vi "Add ECAT Slave from Config.vi"(8 "error in (no error)":errorcluster, 10 "Section Ptr":T4 format="%.0x", 11 "Slave":T1) -> (0 "error out":errorcluster)   [LabVIEW 2020, in "SEECD System Explorer.lvlib"]
uses:
  SEECD System Explorer.lvlib
  <vilib>/NI VeriStand/Custom Device API/Custom Device Item Ref.ctl
  Type Defs/Host - Slave.ctl
  Type Defs/Host - Module.ctl
  Type Defs/IOV Container Contents.ctl
  Includes/Modules.lvlibp/RSI Module/Slot Settings.ctl
  Includes/Modules.lvlibp/RSI Module/Module Models.ctl
  Shared/Globals/Scan Engine GUIDs.vi
  Shared/Globals/String Constants.vi
  Shared/Globals/Property Strings.vi
  Includes/Modules.lvlibp/RSI Module/Class Property Strings.vi
  Includes/Modules.lvlibp/RSI Module/RSI Module.lvclass
  Includes/Modules.lvlibp/RemIO Module/RemIO Module.lvclass
  Shared/SEECD Shared.lvlib
  <vilib>/NI VeriStand/Custom Device API/Custom Device API.lvlib
  Includes/Modules.lvlibp
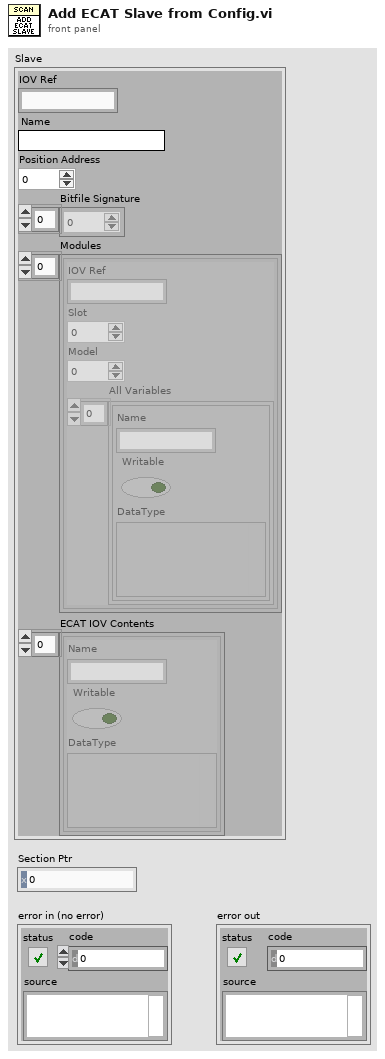
[diagram p1: front panel]
types:
  T1 = typedef "SEECD System Explorer.lvlib/Host - Slave.ctl" = cluster{"IOV Ref":string, "Name":string, "Position Address":u16, "Bitfile Signature":u8[], "Modules":T2[], "ECAT IOV Contents":T3[]}
  T2 = typedef "SEECD System Explorer.lvlib/Host - Module.ctl" = cluster{"IOV Ref":string, "Slot":u32, "Model":u32, "All Variables":T3[]}
  T3 = typedef "SEECD System Explorer.lvlib/IOV Container Contents.ctl" = cluster{"Name":string, "Writable":bool, "DataType":variant}
  T4 = typedef "Custom Device API.lvlib/Custom Device Item Ref.ctl" = u64
  T5 = typedef "Modules.lvlibp/RSI Module.lvclass/Slot Settings.ctl" = cluster{"Slot":u32, "EtherCAT?":bool}
  T6 = typedef "Modules.lvlibp/RSI Module.lvclass/Module Models.ctl" = enum16{"Empty", "NI 9201", "NI 9203", "NI 9205", "NI 9206", "NI 9207", "NI 9208", "NI 9209", "NI 9210", "NI 9211", "NI 9212", "NI 9213", "NI 9214", "NI 9215", "NI 9216", "NI 9217", "NI 9219", "NI 9220", "NI 9221", "NI 9222", "NI 9223", "NI 9224", "NI 9225", "NI 9226", "NI 9227", "NI 9228", "NI 9229", "NI 9233", "NI 9234", "NI 9235", "NI 9236", "NI 9237", "NI 9239", "NI 9242", "NI 9244", "NI 9253", "NI 9263", "NI 9264", "NI 9265", "NI 9266", "NI 9269", "NI 9344", "NI 9350", "NI 9375", "NI 9401", "NI 9402", "NI 9403", "NI 9411", "NI 9421", "NI 9422", "NI 9423", "NI 9425", "NI 9426", "NI 9435", "NI 9436", "NI 9437", "NI 9472", "NI 9474", "NI 9475", "NI 9476", "NI 9477", "NI 9478", "NI 9481", "NI 9482", "NI 9485"}
  T7 = typedef "Modules.lvlibp/Custom Device API.lvlib/Custom Device Item Ref.ctl" = u64
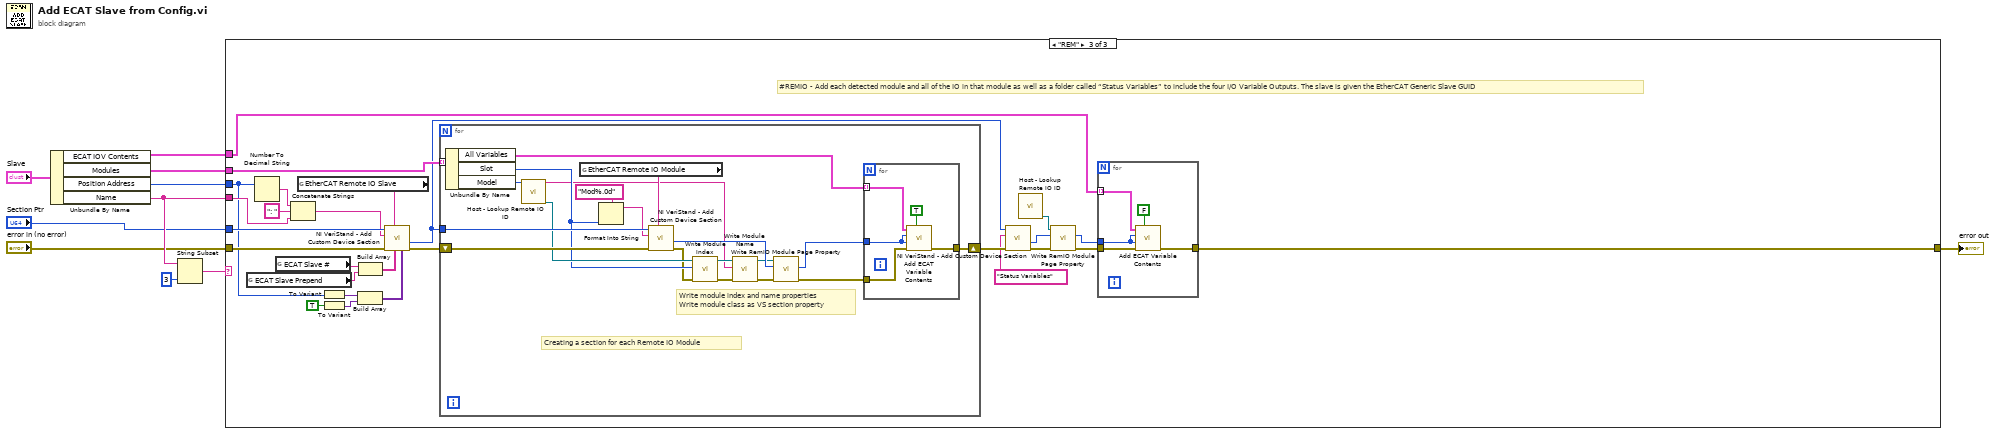
[diagram p0: block diagram]
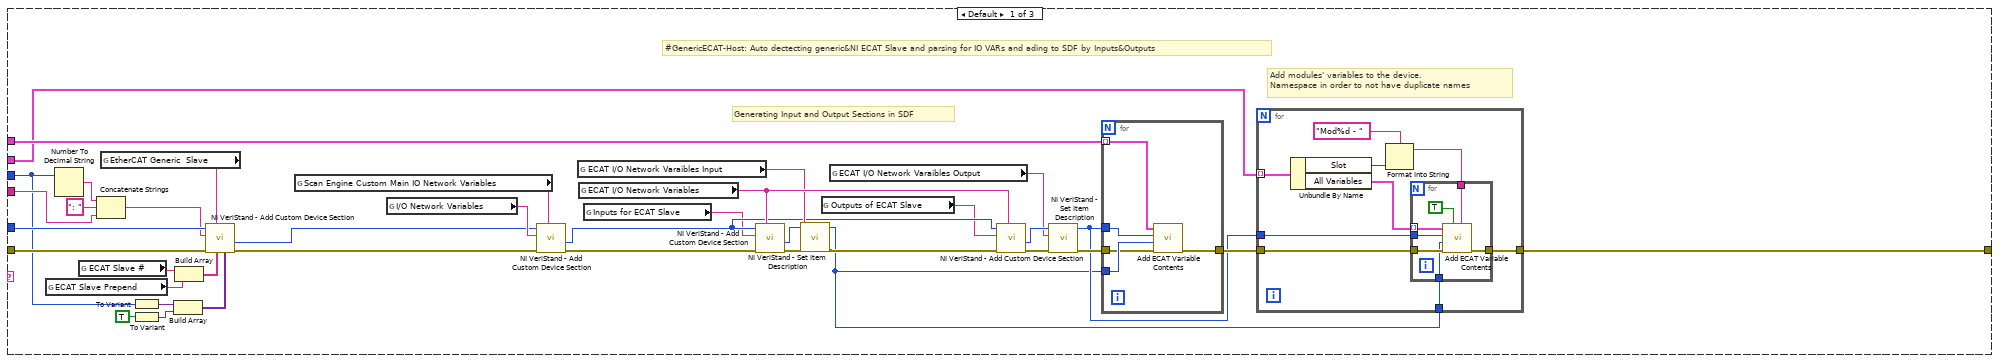
[diagram p2: hidden frame]
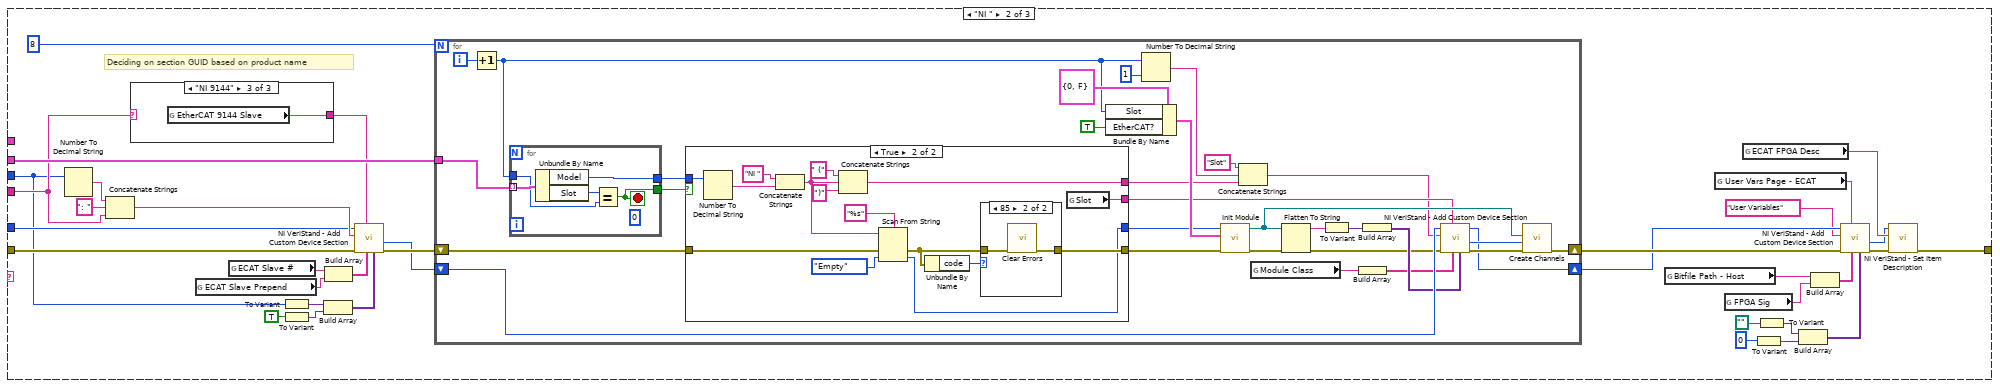
[diagram p3: hidden frame]
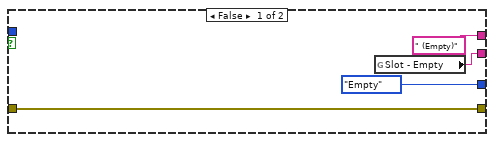
[diagram p4: hidden frame]
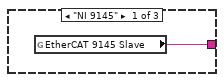
[diagram p6: hidden frame]
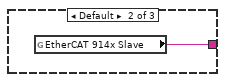
[diagram p7: hidden frame]
diagram:
  n1 = Unbundle By Name("Slave") -> ("ECAT IOV Contents"=w7:T3[], "Modules"=w4:T2[], "Position Address"=w9:u16, "Name"=w10:string)
  n2 = String Subset(string=w10, length (rest)=3 ("Länge (Rest)")) -> (substring=w8:string)  [unwired: 1 in]
  n3 = case shown="\"REM\"" w8 {
    tunnel: "error in (no error)" -> [w33 w88 w182]
    tunnel: w4 -> [w15 w87 w190]
    tunnel: [w13 w86 w188] -> w5
    tunnel: w7 -> [w48 _ w187]
    tunnel: "Section Ptr" -> [w32 w73 w179]
    tunnel: w9 -> [w17 w70 w166]
    tunnel: w10 -> [w20 w72 w169]
    frame Default {
      # "Add modules' variables to the device.\nNamespace in order to not have duplicate names"
      # "#GenericECAT-Host: Auto dectecting generic&NI ECAT Slave and parsing for IO VARs and ading to SDF by Inputs&Outputs"
      # "Generating Input and Output Sections in SDF"
      n4 = global read "Property Strings.vi" "ECAT Slave Prepend"() -> (w24:string)
      n5 = Number To Decimal String(number=w17) -> (decimal integer string=w27:string)  [unwired: 1 in]
      n6 = global read "Property Strings.vi" "ECAT Slave #"() -> (w25:string)
      n7 = Concatenate Strings(w27, ": " ("string"), w20) -> (w29:string)
      n8 = global read "Scan Engine GUIDs.vi" "EtherCAT Generic  Slave"() -> (w30:string)
      n9 = To Variant(anything=w17) -> (Variant=w23:variant)
      n10 = To Variant(anything=TRUE) -> (Variant=w22:variant)
      n11 = Build Array(w23, w22) -> (w19:variant[])
      n12 = Build Array(w25, w24) -> (w26:string[])
      n13 = call <vilib>:"NI VeriStand - Add Custom Device Section.vi"("Property Values"=w19, "Property names"=w26, "GUID (Default Section)"=w30, "error in (no error)"=w33, "Section Name"=w29, "Parent Ref in"=w32) -> ("error out"=w31:errorcluster, "Section Ptr"=w14:T4)  [unwired: 2 in, 2 out]
      n14 = global read "Scan Engine GUIDs.vi" "Scan Engine Custom Main IO Network Variables"() -> (w43:string)
      n15 = global read "Property Strings.vi" "I/O Network Variables"() -> (w36:string)
      n16 = call <vilib>:"NI VeriStand - Add Custom Device Section.vi"("GUID (Default Section)"=w43, "error in (no error)"=w31, "Section Name"=w36, "Parent Ref in"=w14) -> ("error out"=w37:errorcluster, "Section Ptr"=w38:T4)  [unwired: 4 in, 2 out]
      n17 = global read "String Constants.vi" "ECAT I/O Network Varaibles Input"() -> (w39:string)
      n18 = global read "Scan Engine GUIDs.vi" "ECAT I/O Network Variables"() -> (w40:string)
      n19 = global read "Property Strings.vi" "Inputs for ECAT Slave"() -> (w35:string)
      n20 = call <vilib>:"NI VeriStand - Add Custom Device Section.vi"("GUID (Default Section)"=w40, "error in (no error)"=w37, "Section Name"=w35, "Parent Ref in"=w38) -> ("error out"=w47:errorcluster, "Section Ptr"=w42:T4)  [unwired: 4 in, 2 out]
      n21 = call <vilib>:"NI VeriStand - Set Item Description.vi"("error in (no error)"=w47, "Description"=w39, "Item Ref in"=w42) -> ("error out"=w46:errorcluster, "Item Ref out"=w11:T4)  [unwired: 6 in, 1 out]
      n22 = global read "Property Strings.vi" "Outputs of ECAT Slave"() -> (w34:string)
      n23 = global read "String Constants.vi" "ECAT I/O Network Varaibles Output"() -> (w18:string)
      n24 = call <vilib>:"NI VeriStand - Add Custom Device Section.vi"("GUID (Default Section)"=w40, "error in (no error)"=w46, "Section Name"=w34, "Parent Ref in"=w38) -> ("error out"=w45:errorcluster, "Section Ptr"=w41:T4)  [unwired: 4 in, 2 out]
      n25 = call <vilib>:"NI VeriStand - Set Item Description.vi"("error in (no error)"=w45, "Description"=w18, "Item Ref in"=w41) -> ("error out"=w44:errorcluster, "Item Ref out"=w12:T4)  [unwired: 6 in, 1 out]
      n26 = for {
        tunnel: w48 -> [w65] mode=indexing
        tunnel: [w67] -> w16
        tunnel: w44 -> [w66]
        tunnel: w12 -> [w69]
        tunnel: w11 -> [w68]
        n27 = call "Add ECAT Variable Contents.vi"("error in"=w66, "Input Parent Ref in"=w68, "Output Parent Ref in"=w69, "IO Variable Container Contents"=w65) -> ("error out"=w67:errorcluster)  [unwired: 7 in]
      }
      n28 = for {
        tunnel: w16 -> [w51]
        tunnel: w15 -> [w57] mode=indexing
        tunnel: [w53] -> w13
        tunnel: w12 -> [w50]
        tunnel: w11 -> [w49]
        n29 = Unbundle By Name(w57) -> ("Slot"=w56:u32, "All Variables"=w54:T3[])
        n30 = Format Into String(format string="Mod%d - ", w56) -> (resulting string=w52:string)  [unwired: 2 in, 1 out]
        n31 = for {
          tunnel: w54 -> [w64] mode=indexing
          tunnel: [w62] -> w53
          tunnel: w52 -> [w61]
          tunnel: w51 -> [w60]
          tunnel: w50 -> [w59]
          tunnel: w49 -> [w58]
          n32 = call "Add ECAT Variable Contents.vi"("Name Prefix"=w61, "Add Name Property"=TRUE, "error in"=w60, "Input Parent Ref in"=w58, "Output Parent Ref in"=w59, "IO Variable Container Contents"=w64) -> ("error out"=w62:errorcluster)  [unwired: 5 in]
        }
      }
    }
    frame "NI " {
      # "Deciding on section GUID based on product name"
      n33 = Number To Decimal String(number=w70) -> (decimal integer string=w84:string)  [unwired: 1 in]
      n34 = Concatenate Strings(w84, ": " ("string"), w72) -> (w82:string)
      n35 = case shown="\"NI 9144\"" w72 {
        tunnel: [w161 w162 w163] -> w71
        frame "NI 9145" {
          n36 = global read "Scan Engine GUIDs.vi" "EtherCAT 9145 Slave"() -> (w161:string)
        }
        frame Default {
          n37 = global read "Scan Engine GUIDs.vi" "EtherCAT 914x Slave"() -> (w162:string)
        }
        frame "NI 9144" {
          n38 = global read "Scan Engine GUIDs.vi" "EtherCAT 9144 Slave"() -> (w163:string)
        }
      }
      n39 = global read "Property Strings.vi" "ECAT Slave Prepend"() -> (w80:string)
      n40 = global read "Property Strings.vi" "ECAT Slave #"() -> (w79:string)
      n41 = To Variant(anything=w70) -> (Variant=w81:variant)
      n42 = To Variant(anything=TRUE) -> (Variant=w75:variant)
      n43 = Build Array(w81, w75) -> (w77:variant[])
      n44 = Build Array(w79, w80) -> (w78:string[])
      n45 = call <vilib>:"NI VeriStand - Add Custom Device Section.vi"("Property Values"=w77, "Property names"=w78, "GUID (Default Section)"=w71, "Section Name"=w82, "Parent Ref in"=w73) -> ("Section Ptr"=w74:T4)  [unwired: 3 in, 3 out]
      n46 = for {
        N: 8 -> [_]
        shift-right: [w107] -> w99
        shift-left: w88 -> [w113]
        shift-right: [w105] -> w98
        shift-left: w74 -> [w133]
        tunnel: w87 -> [w118]
        i -> [w130]
        n47 = Increment(x=w130) -> (x+1=w117:i32)
        n48 = for {
          tunnel: w118 -> [w160] mode=indexing
          tunnel: w117 -> [w158]
          tunnel: [w157] -> w116
          tunnel: [w156] -> w111
          stop <- w157 stop-if-true
          (unwired) u32 0 ("Model")
          n49 = Unbundle By Name(w160) -> ("Model"=w156:u32, "Slot"=w159:u32)
          n50 = Equal?(x=w159, y=w158) -> (x = y?=w157:bool)
        }
        n51 = case shown="True" w116 {
          tunnel: [" (Empty)" ("Section Name") w139] -> w115
          tunnel: [Module_Models."Empty" ("Module") w146] -> w114
          tunnel: w113 -> [w135 w147]
          tunnel: [w135 w148] -> w112
          tunnel: w111 -> [_ w145]
          tunnel: [w134 w138] -> w106
          frame False {
            n52 = global read "Scan Engine GUIDs.vi" "Slot - Empty"() -> (w134:string)
          }
          frame True {
            n53 = Number To Decimal String(number=w145) -> (decimal integer string=w144:string)  [unwired: 1 in]
            n54 = Concatenate Strings("NI " ("string"), w144) -> (w142:string)
            n55 = Concatenate Strings(" (" ("string"), w142, ")" ("string")) -> (w139:string)
            n56 = Scan From String(format string="%s", input string=w142, error in=w147, default 1=Module_Models."Empty" ("Module")) -> (error out=w149:errorcluster, output 1=w146:T6)  [unwired: 1 in, 2 out]
            n57 = Unbundle By Name(w149) -> ("code"=w150:i32)
            n58 = case shown="85" w150 {
              tunnel: [w153 w154] -> w148
              tunnel: w149 -> [w153 w155]
              frame 0, Default {
              }
              frame 85 {
                n59 = call <vilib>:"Clear Errors.vi"("error in (no error)"=w155) -> ("error out"=w154:errorcluster)  [unwired: 5 in, 1 out]
              }
            }
            n60 = global read "Scan Engine GUIDs.vi" "Slot"() -> (w138:string)
          }
        }
        n61 = Bundle By Name(cluster=T5 {"Slot"=0, "EtherCAT?"=FALSE} ("Slot Settings"), "Slot"=w117, "EtherCAT?"=TRUE) -> (w127:T5)
        n62 = Number To Decimal String(number=w117, width (-)=i16 1) -> (decimal integer string=w132:string)
        n63 = call "Init Module.vi"("error in (no error)"=w112, "Slot Settings"=w127, "Module Model"=w114) -> ("error out"=w122:errorcluster, "RSI Module out"=w108:refnum<class "RSI Module.lvclass">)  [unwired: 7 in]
        n64 = Concatenate Strings("Slot" ("string"), w132, w115) -> (w104:string)
        n65 = global read "Class Property Strings.vi" "Module Class"() -> (w120:string)
        n66 = Flatten To String(anything=w108, error in (no error)=w122) -> (data string=w123:string, error out=w121:errorcluster)  [unwired: 2 in, 1 out]
        n67 = To Variant(anything=w123) -> (Variant=w128:variant)
        n68 = Build Array(w120) -> (w124:string[])
        n69 = Build Array(w128) -> (w129:variant[])
        n70 = call <vilib>:"NI VeriStand - Add Custom Device Section.vi"("Property Values"=w129, "Property names"=w124, "GUID (Default Section)"=w106, "error in (no error)"=w121, "Section Name"=w104, "Parent Ref in"=w133) -> ("error out"=w109:errorcluster, "Section Ptr"=w110:T4, "Parent Ref out"=w105:T4)  [unwired: 2 in, 1 out]
        n71 = call-dynamic "Create Channels.vi"("error in (no error)"=w109, "RSI Module in"=w108, "Parent Ref in"=w110) -> ("error out"=w107:errorcluster)  [unwired: 6 in, 2 out]
      }
      n72 = global read "Property Strings.vi" "Bitfile Path - Host"() -> (w90:string)
      n73 = global read "Scan Engine GUIDs.vi" "User Vars Page - ECAT"() -> (w101:string)
      n74 = global read "Property Strings.vi" "FPGA Sig"() -> (w89:string)
      n75 = global read "String Constants.vi" "ECAT FPGA Desc"() -> (w100:string)
      n76 = To Variant(anything=u32 0 ("ModuleIdent (ECAT)")) -> (Variant=w91:variant)
      n77 = To Variant(anything=path "") -> (Variant=w92:variant)
      n78 = Build Array(w92, w91) -> (w102:variant[])
      n79 = Build Array(w90, w89) -> (w103:string[])
      n80 = call <vilib>:"NI VeriStand - Add Custom Device Section.vi"("Property Values"=w102, "Property names"=w103, "GUID (Default Section)"=w101, "error in (no error)"=w99, "Section Name"="User Variables", "Parent Ref in"=w98) -> ("error out"=w95:errorcluster, "Section Ptr"=w96:T4)  [unwired: 2 in, 2 out]
      n81 = call <vilib>:"NI VeriStand - Set Item Description.vi"("error in (no error)"=w95, "Description"=w100, "Item Ref in"=w96) -> ("error out"=w86:errorcluster)  [unwired: 6 in, 2 out]
    }
    frame "REM" {
      # "#REMIO - Add each detected module and all of the IO in that module as well as a folder called “Status Variables” to include the four I/O Variable Outputs. The slave is given the EtherCAT Generic Slave GUID"
      n82 = global read "Property Strings.vi" "ECAT Slave Prepend"() -> (w173:string)
      n83 = Number To Decimal String(number=w166) -> (decimal integer string=w177:string)  [unwired: 1 in]
      n84 = global read "Property Strings.vi" "ECAT Slave #"() -> (w172:string)
      n85 = Concatenate Strings(w177, ": " ("string"), w169) -> (w175:string)
      n86 = global read "Scan Engine GUIDs.vi" "EtherCAT Remote IO Slave"() -> (w178:string)
      n87 = To Variant(anything=w166) -> (Variant=w174:variant)
      n88 = To Variant(anything=TRUE) -> (Variant=w167:variant)
      n89 = Build Array(w174, w167) -> (w170:variant[])
      n90 = Build Array(w172, w173) -> (w171:string[])
      n91 = call <vilib>:"NI VeriStand - Add Custom Device Section.vi"("Property Values"=w170, "Property names"=w171, "GUID (Default Section)"=w178, "error in (no error)"=w182, "Section Name"=w175, "Parent Ref in"=w179) -> ("error out"=w181:errorcluster, "Section Ptr"=w180:T4)  [unwired: 2 in, 2 out]
      n92 = for {
        shift-right: [w207] -> w189
        shift-left: w181 -> [w210]
        tunnel: w180 -> [w209]
        tunnel: w190 -> [w208] mode=indexing
        # "Write module index and name properties\nWrite module class as VS section property"
        # "Creating a section for each Remote IO Module"
        n93 = Unbundle By Name(w208) -> ("All Variables"=w191:T3[], "Slot"=w204:u32, "Model"=w206:u32)
        n94 = call "Host - Lookup Remote IO ID.vi"("Module ID"=w206) -> ("RemIO Module Out"=w205:refnum<class "RemIO Module.lvclass">, "Module Name"=w193:string)  [unwired: 9 in]
        n95 = global read "Scan Engine GUIDs.vi" "EtherCAT Remote IO Module"() -> (w203:string)
        n96 = Format Into String(format string="Mod%.0d", w204) -> (resulting string=w199:string)  [unwired: 2 in, 1 out]
        n97 = call <vilib>:"NI VeriStand - Add Custom Device Section.vi"("GUID (Default Section)"=w203, "error in (no error)"=w210, "Section Name"=w199, "Parent Ref in"=w209) -> ("error out"=w201:errorcluster, "Section Ptr"=w202:T4)  [unwired: 4 in, 2 out]
        n98 = call-dynamic "Write Module Index.vi"("error in (no error)"=w201, "Module Index"=w204, "RemIO Module in"=w205) -> ("error out"=w196:errorcluster, "RemIO Module out"=w197:refnum<class "RemIO Module.lvclass">)  [unwired: 7 in]
        n99 = call-dynamic "Write Module Name.vi"("error in (no error)"=w196, "Module Name"=w193, "RemIO Module in"=w197) -> ("error out"=w195:errorcluster, "RemIO Module out"=w194:refnum<class "RemIO Module.lvclass">)  [unwired: 7 in]
        n100 = call "Write RemIO Module Page Property.vi"("error in (no error)"=w195, "Node Ptr In"=w202, "RemIO Module"=w194) -> ("error out"=w192:errorcluster, "Node Ptr Out"=w200:T7)  [unwired: 6 in, 1 out]
        n101 = for {
          tunnel: w200 -> [w213]
          tunnel: [w214] -> w207
          tunnel: w192 -> [w215]
          tunnel: w191 -> [w212] mode=indexing
          n102 = call "Add ECAT Variable Contents.vi"("Add Name Property"=TRUE, "error in"=w215, "Input Parent Ref in"=w213, "Output Parent Ref in"=w213, "IO Variable Container Contents"=w212) -> ("error out"=w214:errorcluster)  [unwired: 6 in]
        }
      }
      n103 = call <vilib>:"NI VeriStand - Add Custom Device Section.vi"("error in (no error)"=w189, "Section Name"="Status Variables", "Parent Ref in"=w180) -> ("error out"=w186:errorcluster, "Section Ptr"=w184:T4)  [unwired: 5 in, 2 out]
      n104 = call "Host - Lookup Remote IO ID.vi"() -> ("RemIO Module Out"=w183:refnum<class "RemIO Module.lvclass">)  [unwired: 10 in, 1 out]
      n105 = call "Write RemIO Module Page Property.vi"("error in (no error)"=w186, "Node Ptr In"=w184, "RemIO Module"=w183) -> ("error out"=w185:errorcluster, "Node Ptr Out"=w164:T7)  [unwired: 6 in, 1 out]
      n106 = for {
        tunnel: w187 -> [w218] mode=indexing
        tunnel: w164 -> [w219]
        tunnel: [w216] -> w188
        tunnel: w185 -> [w220]
        n107 = call "Add ECAT Variable Contents.vi"("Add Name Property"=FALSE, "error in"=w220, "Input Parent Ref in"=w219, "Output Parent Ref in"=w219, "IO Variable Container Contents"=w218) -> ("error out"=w216:errorcluster)  [unwired: 6 in]
      }
    }
  }
  "error out" <- w5
